vi "Own20261012_GetBooleanStyleInfo.vi"() -> ()   [LabVIEW 2024]
panel:
  out "state_strings":string[](array[string])
  out "mechanical_action":u32
  out "multiple_strings":bool
  out "error out":errorcluster caption="错误输出"
  out "text":string
  in  "boolean_id":u32
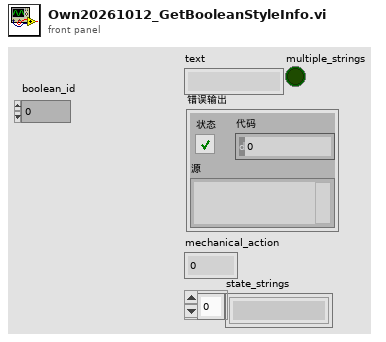
[diagram p1: front panel]
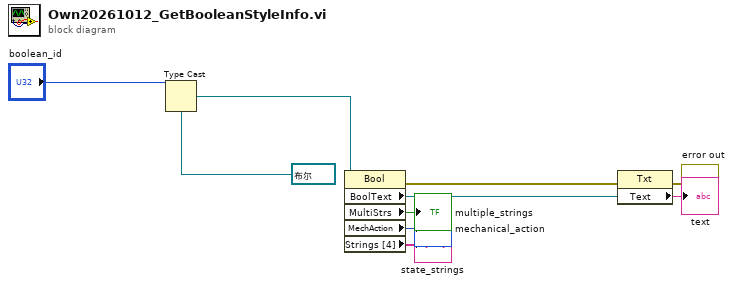
[diagram p0: block diagram]
diagram:
  n1 = Type Cast(type=refnum<vi> refnum ("引用"), x="boolean_id") -> (*(type *) &x=w8:refnum<vi>)
  n2 = property class="Bool"(reference=w8) -> (error out=w6:errorcluster, "BoolText"=w7:refnum<vi>, "MultiStrs"=→"multiple_strings":bool, "MechAction"=→"mechanical_action":u32, "Strings [4]"=→"state_strings":string[])  [unwired: 1 in, 1 out]
  n3 = property class="Txt"(reference=w7, error in=w6) -> (error out=→"error out":errorcluster, "Text"=→"text":string)  [unwired: 1 out]
